vi "Remove Panel from SubPanel.vi"(8 "error in (no error)":errorcluster, 10 "Panel In":refnum<class "Panel.lvclass">, 11 "Manager in":refnum<class "Manager.lvclass">) -> (0 "error out":errorcluster, 2 "Panel":refnum<class "Panel.lvclass">, 3 "Manager out":refnum<class "Manager.lvclass">)   [LabVIEW 2020, in "OOPanel.lvlib" / "Manager.lvclass"]
uses:
  Manager.lvclass
  Panel/Panel.lvclass
  Manager.lvclass/Manager.ctl
  <vilib>/Utility/miscctls.llb/LVMapReplaceAction.ctl
  Visibility State.ctl
  OOPanel.lvlib
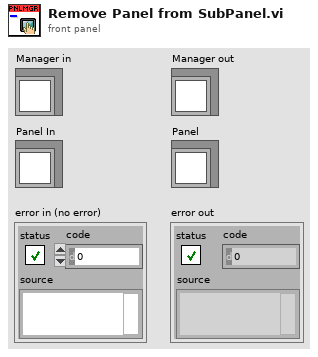
[diagram p1: front panel]
types:
  T1 = typedef "LVMapReplaceAction.ctl" = enum32{"Modify Entry only if found", "Add or Modify Entry", "Delete Entry"}
  T2 = typedef "OOPanel.lvlib/Manager.lvclass/Ref Data.ctl" = cluster{"Created Panels":refnum<class "Panel.lvclass">[], "Subpanel Map":map{refnum<vi>, T3}}
  T3 = typedef "OOPanel.lvlib/Manager.lvclass/Subpanel Data.ctl" = cluster{"Panel":refnum<class "Panel.lvclass">, "Has Panel":bool, "Visible":bool}
  T4 = typedef "OOPanel.lvlib/Visibility State.ctl" = enum16{"Idle", "Closed", "Hidden", "Visible", "Subpanel", "Hidden Subpanel"}
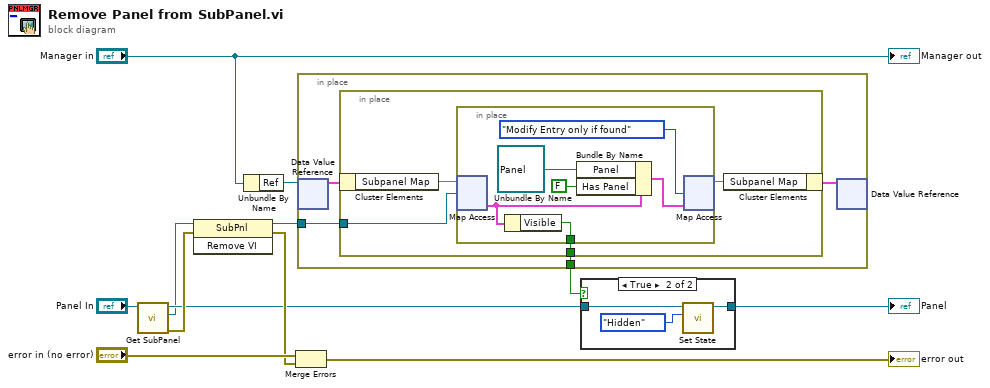
[diagram p0: block diagram]
diagram:
  n1 = call "Get SubPanel.vi"("Panel in"="Panel In") -> ("error out"=w7:errorcluster, "SubPanel"=w2:refnum<vi>, "Panel out"=w4:refnum<class "Panel.lvclass">)  [unwired: 8 in]
  n2 = invoke class="SubPnl" method="Remove VI"(reference=w2, error in=w7) -> (reference out=w8:refnum<vi>, error out=w5:errorcluster)  [unwired: 1 in, 1 out]
  n3 = Unbundle By Name("Manager in") -> ("Ref"=w10:refnum<data-value>)
  n4 = Merge Errors("error in (no error)", w5) -> (→"error out":errorcluster)
  n5 = in-place {
    in-place-border: w8 -> [w14]
    in-place-border: [w13] -> w1
    n6 = in-place-dvr #1(w10) -> (w16:T2)  [unwired: 1 out]
    n7 = in-place {
      in-place-border: w14 -> [w19]
      in-place-border: [w17] -> w13
      n8 = in-place-cluster #2(w16) -> ("Subpanel Map"=w20:map{refnum<vi>, T3})
      n9 = in-place {
        in-place-border: [w21] -> w17
        n10 = in-place-map #3(w20, w19) -> (w22:T3)  [unwired: 1 in, 1 out]
        n11 = Unbundle By Name(w22) -> ("Visible"=w21:bool)
        n12 = Bundle By Name(cluster=w22, "Panel"=refnum<class "Panel.lvclass"> refnum, "Has Panel"=FALSE) -> (w24:T3)
        n13 = in-place-map #3(w24, LVMapReplaceAction."Modify Entry only if found" ("action")) -> (w18:map{refnum<vi>, T3})  [unwired: 2 out]
      }
      n14 = in-place-cluster #2("Subpanel Map"=w18) -> (w15:T2)
    }
    n15 = in-place-dvr #1(w15) -> ()  [unwired: 2 out]
  }
  n16 = case shown="True" w1 {
    tunnel: w4 -> [w27 w30]
    tunnel: [w27 w29] -> w3
    frame False {
      # "Already hidden"
    }
    frame True {
      n17 = call "Set State.vi"("State"=Visibility_State."Hidden", "Panel in"=w30) -> ("Panel out"=w29:refnum<class "Panel.lvclass">)  [unwired: 8 in, 1 out]
    }
  }
  "Panel" <- w3
  "Manager out" <- "Manager in"
